vi "Validate Signed Representation Test Vectors - Round Trip.vi"() -> ()   [LabVIEW 2026, in "Utility.lvlib"]
doc: "Standalone test harness for signed-representation conversion. Replace placeholder actual result controls by wiring outputs from To Signed Representation.vim over each type test vector."
uses:
  Utility.lvlib
  Types/Signed Representation.ctl
  c9b7b341-efd4-42cb-ad51-01ce383bb850.vi
  2017a117-47f3-4693-8c0d-95cb89b6f652.vi
  9f3f59f3-019b-4fd2-a015-fa6ceef6ff24.vi
  3ef9f9ed-9f8b-4c95-a045-f430f47251d7.vi
  d45d5563-1e70-4b2e-af5d-47e39ffbbc8e.vi
  a8733208-4746-4b40-be0a-48a5e9704170.vi
  1785c33c-7975-48b5-9134-d9e0180d661c.vi
  72e02ec1-529b-464a-8c1f-f3d5fb049e43.vi
  c9b7b341-efd4-42cb-ad51-01ce383bb850.vi/fdd2035b-52a6-4314-93d5-e6d0012ea0d5.vi
  c9b7b341-efd4-42cb-ad51-01ce383bb850.vi/d7ddfa2c-0539-47bf-9b9d-3a470632982d.vi
  c9b7b341-efd4-42cb-ad51-01ce383bb850.vi/b8120071-ec88-4802-9c07-9d147ec9c255.vi
  c9b7b341-efd4-42cb-ad51-01ce383bb850.vi/96d3ddf9-193f-4353-8b9f-7b29ff2119cb.vi
  c9b7b341-efd4-42cb-ad51-01ce383bb850.vi/a2043324-c5a4-4327-a6d6-ab77c0f4b7eb.vi
  2017a117-47f3-4693-8c0d-95cb89b6f652.vi/075529c4-3756-4c35-a727-d79a570b4e4b.vi
  2017a117-47f3-4693-8c0d-95cb89b6f652.vi/f2b159a7-3f15-4c07-8087-86d897f3e084.vi
  2017a117-47f3-4693-8c0d-95cb89b6f652.vi/e7f4747e-5a28-4a2e-9592-f11bd74c8d05.vi
  2017a117-47f3-4693-8c0d-95cb89b6f652.vi/dfb42b1f-79ab-4f7c-b389-1108b947dcfb.vi
  2017a117-47f3-4693-8c0d-95cb89b6f652.vi/5f52ec6b-8d9c-4a1b-8cba-4e2f2acbbc65.vi
  2017a117-47f3-4693-8c0d-95cb89b6f652.vi/9402299f-8d08-4b56-b955-c752433d99a7.vi
  2017a117-47f3-4693-8c0d-95cb89b6f652.vi/587ca7da-2917-4b98-b856-e292118fa9d0.vi
  2017a117-47f3-4693-8c0d-95cb89b6f652.vi/d9cf77ad-bfa9-4690-bb58-8188d63c027f.vi
  2017a117-47f3-4693-8c0d-95cb89b6f652.vi/0dbe1b4e-815d-48eb-bf8e-9c4112dc030e.vi
  9f3f59f3-019b-4fd2-a015-fa6ceef6ff24.vi/fdd2035b-52a6-4314-93d5-e6d0012ea0d5.vi
  9f3f59f3-019b-4fd2-a015-fa6ceef6ff24.vi/d7ddfa2c-0539-47bf-9b9d-3a470632982d.vi
  9f3f59f3-019b-4fd2-a015-fa6ceef6ff24.vi/b8120071-ec88-4802-9c07-9d147ec9c255.vi
  9f3f59f3-019b-4fd2-a015-fa6ceef6ff24.vi/96d3ddf9-193f-4353-8b9f-7b29ff2119cb.vi
  9f3f59f3-019b-4fd2-a015-fa6ceef6ff24.vi/a2043324-c5a4-4327-a6d6-ab77c0f4b7eb.vi
  3ef9f9ed-9f8b-4c95-a045-f430f47251d7.vi/075529c4-3756-4c35-a727-d79a570b4e4b.vi
  3ef9f9ed-9f8b-4c95-a045-f430f47251d7.vi/f2b159a7-3f15-4c07-8087-86d897f3e084.vi
  3ef9f9ed-9f8b-4c95-a045-f430f47251d7.vi/e7f4747e-5a28-4a2e-9592-f11bd74c8d05.vi
  3ef9f9ed-9f8b-4c95-a045-f430f47251d7.vi/dfb42b1f-79ab-4f7c-b389-1108b947dcfb.vi
  3ef9f9ed-9f8b-4c95-a045-f430f47251d7.vi/5f52ec6b-8d9c-4a1b-8cba-4e2f2acbbc65.vi
  3ef9f9ed-9f8b-4c95-a045-f430f47251d7.vi/9402299f-8d08-4b56-b955-c752433d99a7.vi
  3ef9f9ed-9f8b-4c95-a045-f430f47251d7.vi/587ca7da-2917-4b98-b856-e292118fa9d0.vi
  3ef9f9ed-9f8b-4c95-a045-f430f47251d7.vi/d9cf77ad-bfa9-4690-bb58-8188d63c027f.vi
  3ef9f9ed-9f8b-4c95-a045-f430f47251d7.vi/0dbe1b4e-815d-48eb-bf8e-9c4112dc030e.vi
  d45d5563-1e70-4b2e-af5d-47e39ffbbc8e.vi/fdd2035b-52a6-4314-93d5-e6d0012ea0d5.vi
  d45d5563-1e70-4b2e-af5d-47e39ffbbc8e.vi/d7ddfa2c-0539-47bf-9b9d-3a470632982d.vi
  d45d5563-1e70-4b2e-af5d-47e39ffbbc8e.vi/b8120071-ec88-4802-9c07-9d147ec9c255.vi
  d45d5563-1e70-4b2e-af5d-47e39ffbbc8e.vi/96d3ddf9-193f-4353-8b9f-7b29ff2119cb.vi
  d45d5563-1e70-4b2e-af5d-47e39ffbbc8e.vi/a2043324-c5a4-4327-a6d6-ab77c0f4b7eb.vi
  a8733208-4746-4b40-be0a-48a5e9704170.vi/075529c4-3756-4c35-a727-d79a570b4e4b.vi
  a8733208-4746-4b40-be0a-48a5e9704170.vi/f2b159a7-3f15-4c07-8087-86d897f3e084.vi
  a8733208-4746-4b40-be0a-48a5e9704170.vi/e7f4747e-5a28-4a2e-9592-f11bd74c8d05.vi
  a8733208-4746-4b40-be0a-48a5e9704170.vi/dfb42b1f-79ab-4f7c-b389-1108b947dcfb.vi
  a8733208-4746-4b40-be0a-48a5e9704170.vi/5f52ec6b-8d9c-4a1b-8cba-4e2f2acbbc65.vi
  a8733208-4746-4b40-be0a-48a5e9704170.vi/9402299f-8d08-4b56-b955-c752433d99a7.vi
  a8733208-4746-4b40-be0a-48a5e9704170.vi/587ca7da-2917-4b98-b856-e292118fa9d0.vi
  a8733208-4746-4b40-be0a-48a5e9704170.vi/d9cf77ad-bfa9-4690-bb58-8188d63c027f.vi
  a8733208-4746-4b40-be0a-48a5e9704170.vi/0dbe1b4e-815d-48eb-bf8e-9c4112dc030e.vi
  1785c33c-7975-48b5-9134-d9e0180d661c.vi/fdd2035b-52a6-4314-93d5-e6d0012ea0d5.vi
  1785c33c-7975-48b5-9134-d9e0180d661c.vi/d7ddfa2c-0539-47bf-9b9d-3a470632982d.vi
  1785c33c-7975-48b5-9134-d9e0180d661c.vi/b8120071-ec88-4802-9c07-9d147ec9c255.vi
  1785c33c-7975-48b5-9134-d9e0180d661c.vi/96d3ddf9-193f-4353-8b9f-7b29ff2119cb.vi
  1785c33c-7975-48b5-9134-d9e0180d661c.vi/a2043324-c5a4-4327-a6d6-ab77c0f4b7eb.vi
  72e02ec1-529b-464a-8c1f-f3d5fb049e43.vi/075529c4-3756-4c35-a727-d79a570b4e4b.vi
  72e02ec1-529b-464a-8c1f-f3d5fb049e43.vi/f2b159a7-3f15-4c07-8087-86d897f3e084.vi
  72e02ec1-529b-464a-8c1f-f3d5fb049e43.vi/e7f4747e-5a28-4a2e-9592-f11bd74c8d05.vi
  72e02ec1-529b-464a-8c1f-f3d5fb049e43.vi/dfb42b1f-79ab-4f7c-b389-1108b947dcfb.vi
  72e02ec1-529b-464a-8c1f-f3d5fb049e43.vi/5f52ec6b-8d9c-4a1b-8cba-4e2f2acbbc65.vi
  72e02ec1-529b-464a-8c1f-f3d5fb049e43.vi/9402299f-8d08-4b56-b955-c752433d99a7.vi
  72e02ec1-529b-464a-8c1f-f3d5fb049e43.vi/587ca7da-2917-4b98-b856-e292118fa9d0.vi
  72e02ec1-529b-464a-8c1f-f3d5fb049e43.vi/d9cf77ad-bfa9-4690-bb58-8188d63c027f.vi
  72e02ec1-529b-464a-8c1f-f3d5fb049e43.vi/0dbe1b4e-815d-48eb-bf8e-9c4112dc030e.vi
  c9b7b341-efd4-42cb-ad51-01ce383bb850.vi/b8120071-ec88-4802-9c07-9d147ec9c255.vi/8ccb98a6-deb9-4b5a-be05-054c1c212d54.vi
  c9b7b341-efd4-42cb-ad51-01ce383bb850.vi/b8120071-ec88-4802-9c07-9d147ec9c255.vi/f171c548-4dcc-4c0c-949b-fc0df33543c2.vi
  c9b7b341-efd4-42cb-ad51-01ce383bb850.vi/b8120071-ec88-4802-9c07-9d147ec9c255.vi/d8adcdbd-60f3-48f3-8f6a-253ba0c2f91d.vi
  c9b7b341-efd4-42cb-ad51-01ce383bb850.vi/b8120071-ec88-4802-9c07-9d147ec9c255.vi/e61c01d5-f4be-4974-af39-63853a8697d8.vi
  c9b7b341-efd4-42cb-ad51-01ce383bb850.vi/96d3ddf9-193f-4353-8b9f-7b29ff2119cb.vi/8ccb98a6-deb9-4b5a-be05-054c1c212d54.vi
  c9b7b341-efd4-42cb-ad51-01ce383bb850.vi/96d3ddf9-193f-4353-8b9f-7b29ff2119cb.vi/f171c548-4dcc-4c0c-949b-fc0df33543c2.vi
  c9b7b341-efd4-42cb-ad51-01ce383bb850.vi/96d3ddf9-193f-4353-8b9f-7b29ff2119cb.vi/d8adcdbd-60f3-48f3-8f6a-253ba0c2f91d.vi
  c9b7b341-efd4-42cb-ad51-01ce383bb850.vi/96d3ddf9-193f-4353-8b9f-7b29ff2119cb.vi/e61c01d5-f4be-4974-af39-63853a8697d8.vi
  9f3f59f3-019b-4fd2-a015-fa6ceef6ff24.vi/b8120071-ec88-4802-9c07-9d147ec9c255.vi/8ccb98a6-deb9-4b5a-be05-054c1c212d54.vi
  9f3f59f3-019b-4fd2-a015-fa6ceef6ff24.vi/b8120071-ec88-4802-9c07-9d147ec9c255.vi/f171c548-4dcc-4c0c-949b-fc0df33543c2.vi
  9f3f59f3-019b-4fd2-a015-fa6ceef6ff24.vi/b8120071-ec88-4802-9c07-9d147ec9c255.vi/d8adcdbd-60f3-48f3-8f6a-253ba0c2f91d.vi
  9f3f59f3-019b-4fd2-a015-fa6ceef6ff24.vi/b8120071-ec88-4802-9c07-9d147ec9c255.vi/e61c01d5-f4be-4974-af39-63853a8697d8.vi
  9f3f59f3-019b-4fd2-a015-fa6ceef6ff24.vi/96d3ddf9-193f-4353-8b9f-7b29ff2119cb.vi/8ccb98a6-deb9-4b5a-be05-054c1c212d54.vi
  9f3f59f3-019b-4fd2-a015-fa6ceef6ff24.vi/96d3ddf9-193f-4353-8b9f-7b29ff2119cb.vi/f171c548-4dcc-4c0c-949b-fc0df33543c2.vi
  9f3f59f3-019b-4fd2-a015-fa6ceef6ff24.vi/96d3ddf9-193f-4353-8b9f-7b29ff2119cb.vi/d8adcdbd-60f3-48f3-8f6a-253ba0c2f91d.vi
  9f3f59f3-019b-4fd2-a015-fa6ceef6ff24.vi/96d3ddf9-193f-4353-8b9f-7b29ff2119cb.vi/e61c01d5-f4be-4974-af39-63853a8697d8.vi
  d45d5563-1e70-4b2e-af5d-47e39ffbbc8e.vi/b8120071-ec88-4802-9c07-9d147ec9c255.vi/8ccb98a6-deb9-4b5a-be05-054c1c212d54.vi
  d45d5563-1e70-4b2e-af5d-47e39ffbbc8e.vi/b8120071-ec88-4802-9c07-9d147ec9c255.vi/f171c548-4dcc-4c0c-949b-fc0df33543c2.vi
  d45d5563-1e70-4b2e-af5d-47e39ffbbc8e.vi/b8120071-ec88-4802-9c07-9d147ec9c255.vi/d8adcdbd-60f3-48f3-8f6a-253ba0c2f91d.vi
  d45d5563-1e70-4b2e-af5d-47e39ffbbc8e.vi/b8120071-ec88-4802-9c07-9d147ec9c255.vi/e61c01d5-f4be-4974-af39-63853a8697d8.vi
  d45d5563-1e70-4b2e-af5d-47e39ffbbc8e.vi/96d3ddf9-193f-4353-8b9f-7b29ff2119cb.vi/8ccb98a6-deb9-4b5a-be05-054c1c212d54.vi
  d45d5563-1e70-4b2e-af5d-47e39ffbbc8e.vi/96d3ddf9-193f-4353-8b9f-7b29ff2119cb.vi/f171c548-4dcc-4c0c-949b-fc0df33543c2.vi
  d45d5563-1e70-4b2e-af5d-47e39ffbbc8e.vi/96d3ddf9-193f-4353-8b9f-7b29ff2119cb.vi/d8adcdbd-60f3-48f3-8f6a-253ba0c2f91d.vi
  d45d5563-1e70-4b2e-af5d-47e39ffbbc8e.vi/96d3ddf9-193f-4353-8b9f-7b29ff2119cb.vi/e61c01d5-f4be-4974-af39-63853a8697d8.vi
  1785c33c-7975-48b5-9134-d9e0180d661c.vi/b8120071-ec88-4802-9c07-9d147ec9c255.vi/8ccb98a6-deb9-4b5a-be05-054c1c212d54.vi
  1785c33c-7975-48b5-9134-d9e0180d661c.vi/b8120071-ec88-4802-9c07-9d147ec9c255.vi/f171c548-4dcc-4c0c-949b-fc0df33543c2.vi
  1785c33c-7975-48b5-9134-d9e0180d661c.vi/b8120071-ec88-4802-9c07-9d147ec9c255.vi/d8adcdbd-60f3-48f3-8f6a-253ba0c2f91d.vi
  1785c33c-7975-48b5-9134-d9e0180d661c.vi/b8120071-ec88-4802-9c07-9d147ec9c255.vi/e61c01d5-f4be-4974-af39-63853a8697d8.vi
  1785c33c-7975-48b5-9134-d9e0180d661c.vi/96d3ddf9-193f-4353-8b9f-7b29ff2119cb.vi/8ccb98a6-deb9-4b5a-be05-054c1c212d54.vi
  1785c33c-7975-48b5-9134-d9e0180d661c.vi/96d3ddf9-193f-4353-8b9f-7b29ff2119cb.vi/f171c548-4dcc-4c0c-949b-fc0df33543c2.vi
  1785c33c-7975-48b5-9134-d9e0180d661c.vi/96d3ddf9-193f-4353-8b9f-7b29ff2119cb.vi/d8adcdbd-60f3-48f3-8f6a-253ba0c2f91d.vi
  1785c33c-7975-48b5-9134-d9e0180d661c.vi/96d3ddf9-193f-4353-8b9f-7b29ff2119cb.vi/e61c01d5-f4be-4974-af39-63853a8697d8.vi
panel:
  in  "u64 expected encoded":u64[](array[numeric])=[0, 1, 18446744073709551615, 9223372036854775808, 9223372036854775807, 1, 0, 9223372036854775809, 18446744073709551615, 1, 0, 18446744073709551614, 9223372036854775808] format="%016x"
  in  "u32 expected encoded":u32[](array[numeric])=[0, 1, 4294967295, 2147483648, 2147483647, 1, 0, 2147483649, 4294967295, 1, 0, 4294967294, 2147483648] format="%08x"
  in  "u16 expected encoded":u16[](array[numeric])=[0, 1, 65535, 32768, 32767, 1, 0, 32769, 65535, 1, 0, 65534, 32768] format="%04x"
  in  "expected valid":bool[](array[boolean])=[TRUE, TRUE, TRUE, TRUE, TRUE, TRUE, TRUE, TRUE, FALSE, TRUE, TRUE, TRUE, FALSE]
  in  "u8 expected encoded":u8[](array[numeric])=[0, 1, 255, 128, 127, 1, 0, 129, 255, 1, 0, 254, 128] format="%02x"
  out "all tests pass?":bool
  out "i64 pass?":bool
  in  "i64 test values":i64[](array[numeric])=[0, 1, -1, 0, -1, 1, 0, -1, -9223372036854775808, 1, 0, -1, -9223372036854775808]
  out "i32 pass?":bool
  in  "i32 test values":i32[](array[numeric])=[0, 1, -1, 0, -1, 1, 0, -1, -2147483648, 1, 0, -1, -2147483648]
  out "i16 pass?":bool
  in  "i16 test values":i16[](array[numeric])=[0, 1, -1, 0, -1, 1, 0, -1, -32768, 1, 0, -1, -32768]
  out "i8 pass?":bool
  in  "test encodings":T1[](array[typedef])=[enum."Two's Complement", enum."Two's Complement", enum."Two's Complement", enum."Offset Binary", enum."Offset Binary", enum."Sign-Magnitude", enum."Sign-Magnitude", enum."Sign-Magnitude", enum."Sign-Magnitude", enum."Ones' Complement", enum."Ones' Complement", enum."Ones' Complement", enum."Ones' Complement"]
  in  "i8 test values":i8[](array[numeric])=[0, 1, -1, 0, -1, 1, 0, -1, -128, 1, 0, -1, -128]
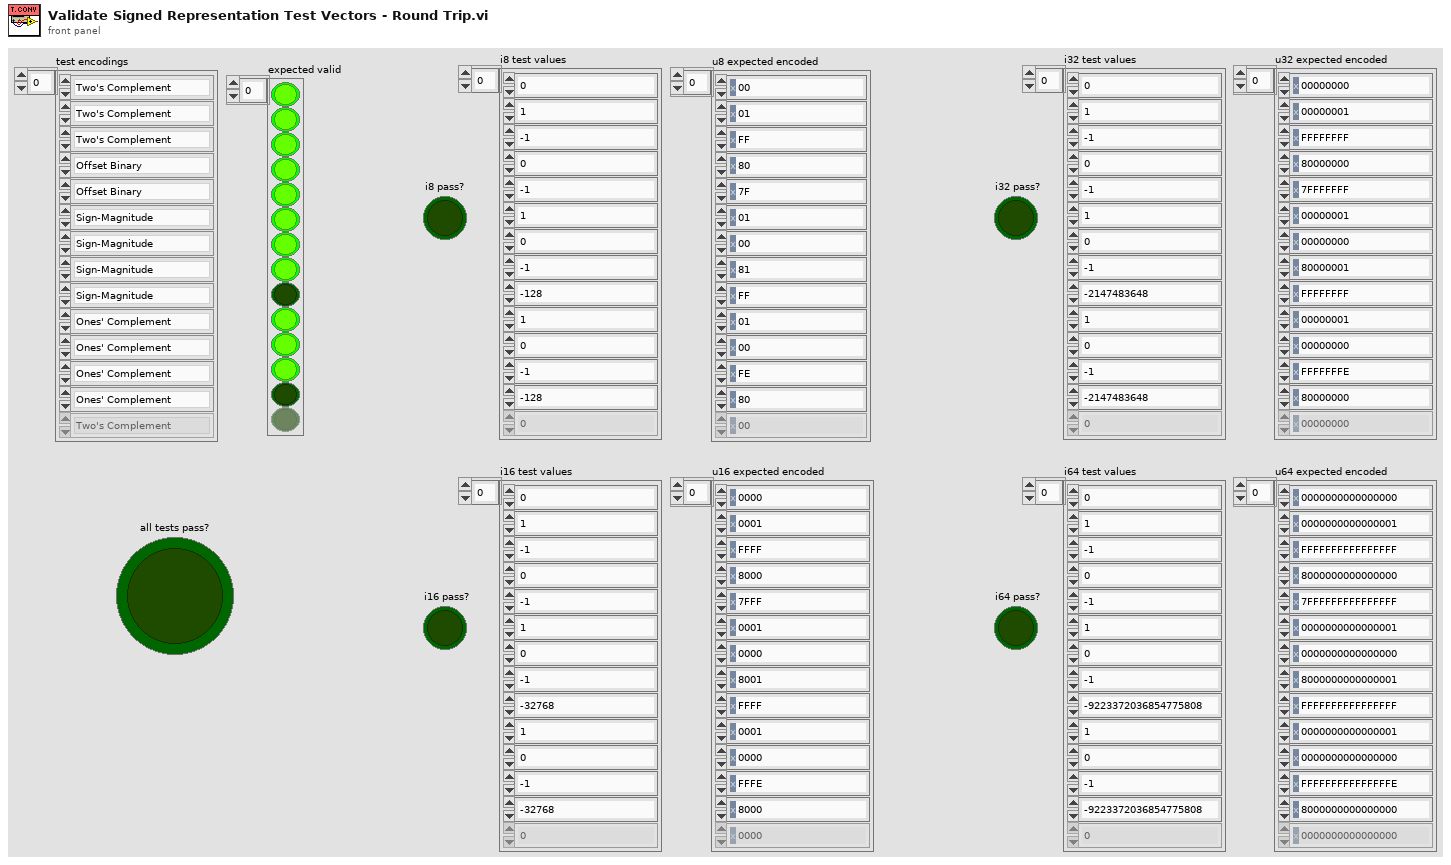
[diagram p1: front panel]
types:
  T1 = typedef "Utility.lvlib/Signed Representation.ctl" = enum16{"Two's Complement", "Offset Binary", "Sign-Magnitude", "Ones' Complement"}
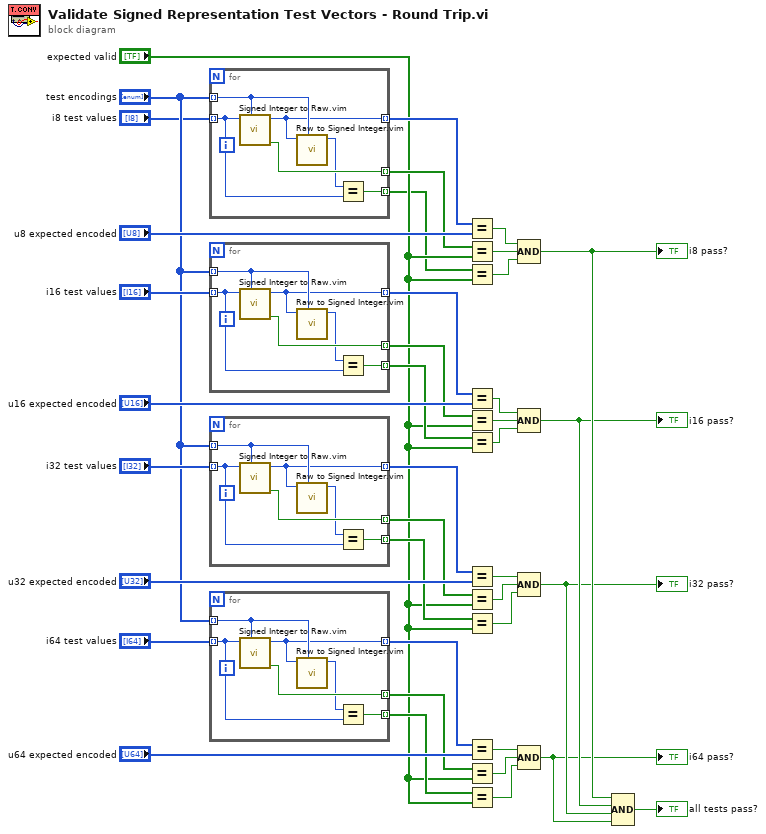
[diagram p0: block diagram]
diagram:
  n1 = for {
    tunnel: "test encodings" -> [w44] mode=indexing
    tunnel: "i8 test values" -> [w41] mode=indexing
    tunnel: [w42] -> w5 mode=indexing
    tunnel: [w45] -> w4 mode=indexing
    tunnel: [w40] -> w1 mode=indexing
    n2 = call "Signed Integer to Raw.vim"("Signed representation"=w44, "Value in"=w41) -> ("Valid?"=w45:bool, "Value (raw)"=w42:u8)  [unwired: 8 in]
    n3 = call "Raw to Signed Integer.vim"("Signed representation"=w44, "Value (raw)"=w42) -> ("Value out"=w43:i8)  [unwired: 8 in, 1 out]
    n4 = Equal?(x=w43, y=w41) -> (x = y?=w40:bool)
  }
  n5 = for {
    tunnel: "test encodings" -> [w50] mode=indexing
    tunnel: "i16 test values" -> [w47] mode=indexing
    tunnel: [w48] -> w11 mode=indexing
    tunnel: [w51] -> w10 mode=indexing
    tunnel: [w46] -> w8 mode=indexing
    n6 = call "Signed Integer to Raw.vim"("Signed representation"=w50, "Value in"=w47) -> ("Valid?"=w51:bool, "Value (raw)"=w48:u16)  [unwired: 8 in]
    n7 = call "Raw to Signed Integer.vim"("Signed representation"=w50, "Value (raw)"=w48) -> ("Value out"=w49:i16)  [unwired: 8 in, 1 out]
    n8 = Equal?(x=w49, y=w47) -> (x = y?=w46:bool)
  }
  n9 = for {
    tunnel: "test encodings" -> [w56] mode=indexing
    tunnel: "i32 test values" -> [w53] mode=indexing
    tunnel: [w54] -> w16 mode=indexing
    tunnel: [w57] -> w15 mode=indexing
    tunnel: [w52] -> w14 mode=indexing
    n10 = call "Signed Integer to Raw.vim"("Signed representation"=w56, "Value in"=w53) -> ("Valid?"=w57:bool, "Value (raw)"=w54:u32)  [unwired: 8 in]
    n11 = call "Raw to Signed Integer.vim"("Signed representation"=w56, "Value (raw)"=w54) -> ("Value out"=w55:i32)  [unwired: 8 in, 1 out]
    n12 = Equal?(x=w55, y=w53) -> (x = y?=w52:bool)
  }
  n13 = for {
    tunnel: "test encodings" -> [w62] mode=indexing
    tunnel: "i64 test values" -> [w59] mode=indexing
    tunnel: [w60] -> w21 mode=indexing
    tunnel: [w63] -> w20 mode=indexing
    tunnel: [w58] -> w19 mode=indexing
    n14 = call "Signed Integer to Raw.vim"("Signed representation"=w62, "Value in"=w59) -> ("Valid?"=w63:bool, "Value (raw)"=w60:u64)  [unwired: 8 in]
    n15 = call "Raw to Signed Integer.vim"("Signed representation"=w62, "Value (raw)"=w60) -> ("Value out"=w61:i64)  [unwired: 8 in, 1 out]
    n16 = Equal?(x=w61, y=w59) -> (x = y?=w58:bool)
  }
  n17 = Equal?(x=w5, y="u8 expected encoded") -> (x = y?=w38:bool)
  n18 = Equal?(x=w4, y="expected valid") -> (x = y?=w37:bool)
  n19 = Equal?(x=w1, y="expected valid") -> (x = y?=w3:bool)
  n20 = Equal?(x=w11, y="u16 expected encoded") -> (x = y?=w35:bool)
  n21 = Equal?(x=w10, y="expected valid") -> (x = y?=w34:bool)
  n22 = Equal?(x=w8, y="expected valid") -> (x = y?=w9:bool)
  n23 = Equal?(x=w16, y="u32 expected encoded") -> (x = y?=w32:bool)
  n24 = Equal?(x=w15, y="expected valid") -> (x = y?=w31:bool)
  n25 = Equal?(x=w14, y="expected valid") -> (x = y?=w13:bool)
  n26 = Equal?(x=w21, y="u64 expected encoded") -> (x = y?=w29:bool)
  n27 = Equal?(x=w20, y="expected valid") -> (x = y?=w28:bool)
  n28 = Equal?(x=w19, y="expected valid") -> (x = y?=w18:bool)
  n29 = Compound Arithmetic op=AND(w38, w37, w3) -> (w26:bool)
  "i8 pass?" <- w26
  n30 = Compound Arithmetic op=AND(w35, w34, w9) -> (w25:bool)
  "i16 pass?" <- w25
  n31 = Compound Arithmetic op=AND(w32, w31, w13) -> (w24:bool)
  "i32 pass?" <- w24
  n32 = Compound Arithmetic op=AND(w29, w28, w18) -> (w23:bool)
  "i64 pass?" <- w23
  n33 = Compound Arithmetic op=AND(w26, w25, w24, w23) -> (→"all tests pass?":bool)
